vi "main.vi"() -> ()   [LabVIEW 2011]
doc: "Main vi of the DCV Build Up Method."
uses:
  Measurement Setting.ctl
  <vilib>/Utility/error.llb/DialogType.ctl
  <vilib>/Utility/NIReport.llb/NI_report.lvclass
  <vilib>/addons/_office/excel.llb/Excel Easy Table (str).vi
  <vilib>/Analysis/NI_AALBase.lvlib
  <vilib>/addons/_office/NI_ReportGenerationToolkit.lvlib
panel:
  in  "Stop all":bool
  out "credentials":string="method by MSL, labview implementation by ÈMI\ncontact:\nm.early@irl.cri.nz, \nmsira@cmi.cz"
  in  "Wait before start [s]:":i32=60
  out "no of templates":i32 caption="of"
  out "current template no":i32 caption="Now running template number:"
  in  "List of templates paths:":path[](array[path])=[path ""]
  out "error out":errorcluster
  out "Standard deviation:":dbl format="%_3pV"
  out "Mean:":dbl format="%_8pV"
  out "Current excel row:":i32
  in  "Source X\n(Fluke calibrator)":refnum<visa-resource-name>="GPIB0::5::INSTR"
  in  "Voltmeter\n(Agilent 3458)":refnum<visa-resource-name>="GPIB0::22::INSTR"
  in  "Source Ref\n(Datron calibrator)":refnum<visa-resource-name>="GPIB0::19::INSTR"
  in  "End row Cell\nposition:":cluster{"row":i32, "column":i32}={"row"=3, "column"=3}
  in  "Start row Cell\nposition:":cluster{"row":i32, "column":i32}={"row"=3, "column"=1}
  out "Current excel template path:":path
  in  "Stop":bool
  # "DCV Build Up Method"
  # "Last voltmeter reading:"
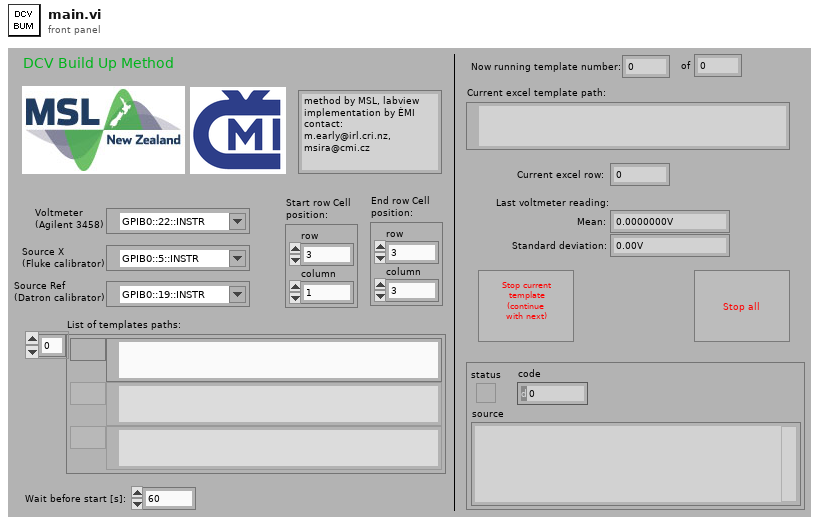
[diagram p1: front panel]
types:
  T1 = typedef "Measurement Setting.ctl" = cluster{"Source X Range":dbl, "Source X Setting":dbl, "Source S Ref Setting":dbl, "Source S Zero Range":dbl, "Voltmeter Nominal Reading":dbl, "No. Readings":dbl, "Delay ms":dbl}
  T2 = typedef "DialogType.ctl" = u16
  T3 = typedef "Measurement References.ctl" = cluster{"Voltmeter VISA":refnum<visa-resource-name>, "Voltmeter error":errorcluster, "Source Ref VISA":refnum<visa-resource-name>, "Source Ref error":errorcluster, "Source X VISA":refnum<visa-resource-name>, "Source X error":errorcluster, "Excel template":refnum<class "NI_report.lvclass">, "Excel template error":errorcluster, "Csv filename":path}
  T4 = cluster{"source x range":string, "source ref range":string, "voltmeter range":string, "voltmeter readings":dbl[], "voltmeter temperature":string}
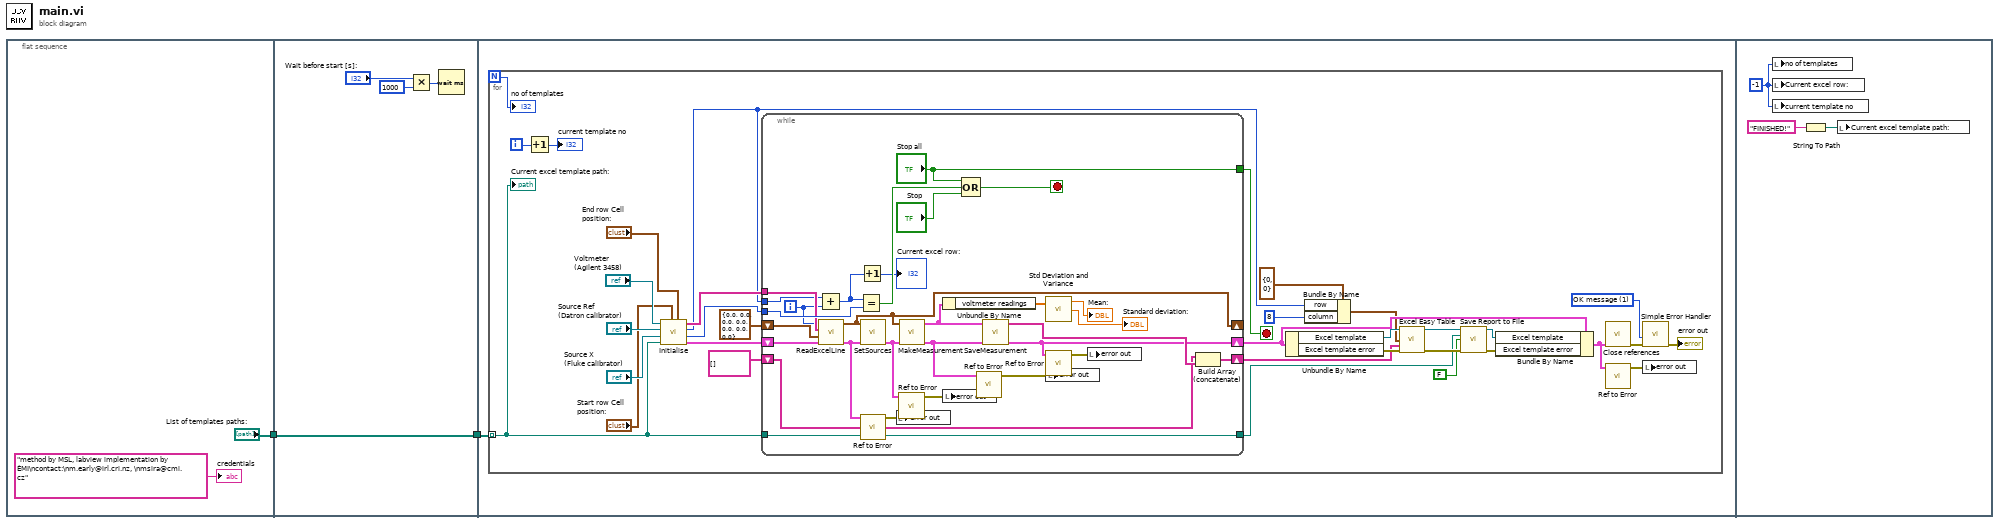
[diagram p0: block diagram]
diagram:
  n1 = flat-sequence {
    tunnel: ["List of templates paths:"] -> w1
    tunnel: [w8] -> w2
    tunnel: w1 -> [w8]
    tunnel: w2 -> [w9]
    frame #0 {
      "credentials" <- "method by MSL, labview implementation by ÈMI\ncontact:\nm.early@irl.cri.nz, \nmsira@cmi.cz" ("String")
    }
    frame #1 {
      n2 = Multiply(x="Wait before start [s]:", y=1000) -> (x*y=w5:i32)
      n3 = Wait (ms)(milliseconds to wait=w5) -> ()  [unwired: 1 out]
    }
    frame #2 {
      n4 = for {
        N -> [w13]
        tunnel: w9 -> [w16] mode=indexing
        i -> [w12]
        stop <- w10 stop-if-true
        w35 = T2 1 items=["no dialog", "OK message", "continue or stop message", "OK message + warnings", "continue/stop + warnings"] ("type of dialog (OK msg:1)")
        n5 = Increment(x=w12) -> (x+1=→"current template no":i32)
        n6 = call "Initialise.vi"("End row Cell position:"="End row Cell\nposition:", "Start row Cell position:"="Start row Cell\nposition:", "Excel template path"=w16, "Source X"="Source X\n(Fluke calibrator)", "Source Ref"="Source Ref\n(Datron calibrator)", "Voltmeter"="Voltmeter\n(Agilent 3458)") -> ("references"=w37:T3, "end row"=w40:i32, "start row"=w18:i32, "measurement settings"=w33:string[][])  [unwired: 2 in]
        n7 = while {
          tunnel: w40 -> [w72]
          shift-right: [w45] -> w25
          shift-left: w37 -> [w68]
          tunnel: w16 -> [w57]
          tunnel: w33 -> [w62]
          tunnel: w18 -> [w56]
          shift-right: [w59] -> w20
          shift-left: string[][] [] -> [w58]
          tunnel: [w57] -> w23
          shift-right: [w53] -> _
          shift-left: T1 {"Source X Range"=0.0, "Source X Setting"=0.0, "Source S Ref Setting"=0.0, "Source S Zero Range"=0.0, "Voltmeter Nominal Reading"=0.0, "No. Readings"=0.0, "Delay ms"=0.0} ("measurement setting") -> [w54]
          tunnel: ["Stop all"] -> w10
          i -> [w61]
          stop <- w69 stop-if-true
          n8 = Add(x=w56, y=w61) -> (x+y=w55:i32)
          n9 = call "ReadExcelLine.vi"("references"=w68, "previous setting"=w54, "measurement settings"=w62, "row number"=w61) -> ("references out"=w52:T3, "measurement setting"=w53:T1)  [unwired: 5 in, 1 out]
          n10 = Equal?(x=w55, y=w72) -> (x = y?=w71:bool)
          n11 = Increment(x=w55) -> (x+1=→"Current excel row:":i32)
          n12 = call "SetSources.vi"("references"=w52, "measurement setting"=w53) -> ("references out"=w47:T3)  [unwired: 9 in]
          n13 = call "Ref to Error.vi"("references"=w52) -> ("error out"=w51:errorcluster)  [unwired: 10 in]
          n14 = local write "error out"(w51) -> ()
          n15 = call "Ref to Error.vi"("references"=w47) -> ("error out"=w50:errorcluster)  [unwired: 10 in]
          n16 = call "MakeMeasurement.vi"("references"=w47, "measurement setting"=w53) -> ("references out"=w46:T3, "measurement"=w67:T4)  [unwired: 8 in]
          n17 = Unbundle By Name(w67) -> ("voltmeter readings"=w66:dbl[])
          n18 = local write "error out"(w50) -> ()
          n19 = Compound Arithmetic op=OR("Stop all", w71, "Stop") -> (w69:bool)
          n20 = call "Ref to Error.vi"("references"=w46) -> ("error out"=w49:errorcluster)  [unwired: 10 in]
          n21 = call "SaveMeasurement.vi"("references"=w46, "measurement"=w67) -> ("references out"=w45:T3, "data"=w60:string[])  [unwired: 8 in]
          n22 = call <vilib>:"Std Deviation and Variance.vi"("X"=w66) -> ("mean"=→"Mean:":dbl, "standard deviation"=→"Standard deviation:":dbl)  [unwired: 1 in, 1 out]
          n23 = call "Ref to Error.vi"("references"=w45) -> ("error out"=w48:errorcluster)  [unwired: 10 in]
          n24 = local write "error out"(w49) -> ()
          n25 = local write "error out"(w48) -> ()
          n26 = Build Array (concatenate)(w58, w60) -> (w59:string[][])
        }
        n27 = Unbundle By Name(w25) -> ("Excel template"=w28:refnum<class "NI_report.lvclass">, "Excel template error"=w29:errorcluster)
        n28 = Bundle By Name(cluster=cluster{"row":i32, "column":i32} {"row"=0, "column"=0} ("start (0, 0)"), "row"=w18, "column"=8) -> (w19:cluster{"row":i32, "column":i32})
        n29 = call-poly <vilib>:"Excel Easy Table.vi"("report in"=w28, "start (0, 0)"=w19, "text data"=w20, "error in (no error)"=w29) -> ("report out"=w31:refnum<class "NI_report.lvclass">, "error out"=w30:errorcluster)  [unwired: 7 in, 3 out]
        n30 = call-dynamic "Save Report to File.vi"("report in"=w31, "report file path"=w23, "prompt to replace? (F)"=FALSE, "error in (no error)"=w30) -> ("report out"=w26:refnum<class "NI_report.lvclass">, "error out"=w27:errorcluster)  [unwired: 10 in]
        n31 = Bundle By Name(cluster=w25, "Excel template"=w26, "Excel template error"=w27) -> (w14:T3)
        n32 = call "Close references.vi"("references"=w14) -> ("error out"=w36:errorcluster)  [unwired: 10 in]
        n33 = call "Ref to Error.vi"("references"=w14) -> ("error out"=w15:errorcluster)  [unwired: 10 in]
        n34 = call <vilib>:"Simple Error Handler.vi"("type of dialog (OK msg:1)"=w35, "error in (no error)"=w36) -> ("error out"=→"error out":errorcluster)  [unwired: 3 in, 4 out]
        n35 = local write "error out"(w15) -> ()
        "Current excel template path:" <- w16
        "no of templates" <- w13
      }
    }
    frame #3 {
      w75 = -1 ("current template no")
      n36 = local write "no of templates"(w75) -> ()
      n37 = local write "Current excel row:"(w75) -> ()
      n38 = local write "current template no"(w75) -> ()
      n39 = String To Path(string="FINISHED!") -> (path=w73:path)
      n40 = local write "Current excel template path:"(w73) -> ()
    }
  }
